vi "ASK Main.vi"() -> ()   [LabVIEW 2026]
panel:
  out "Detected Energy":dbl[](array[numeric])
  out "Recovered Binary Signal":dbl[](array[numeric])
  out "ASK Modulated Signal":dbl[](graph)
  out "Baseband Signal":dbl[](graph)
  in  "Detection Threshold":dbl
  in  "Carrier Amplitude(A)":dbl
  in  "Carrier Frequency(fc)":dbl
  in  "Bit Rate(Rb)":dbl
  in  "Sampling Frequency(Fs)":dbl
  in  "Binary Input":i32[](array[numeric])
  # ".1"
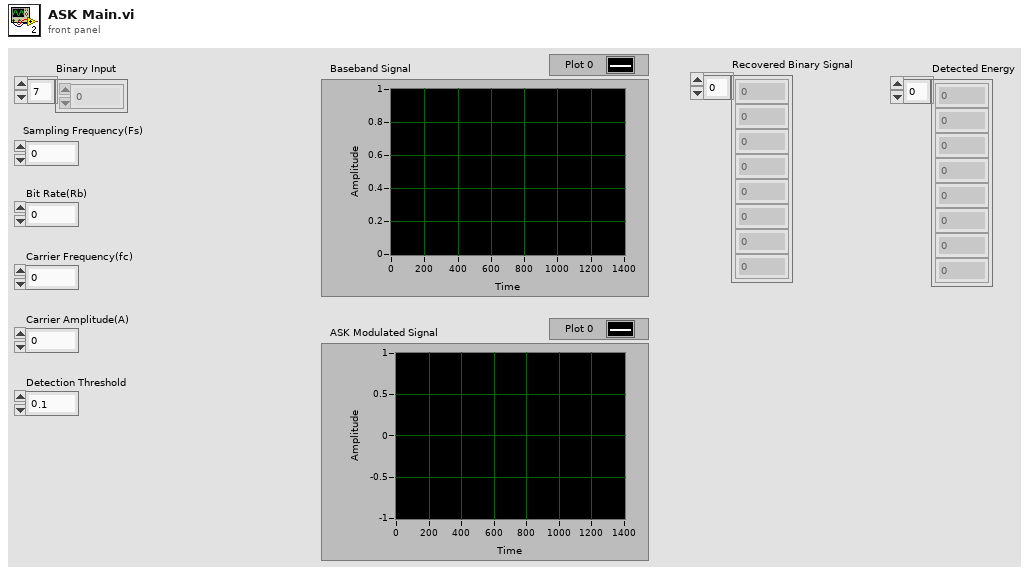
[diagram p1: front panel]
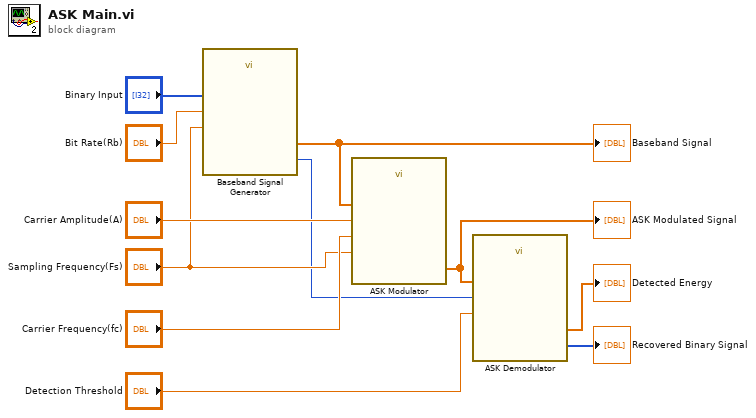
[diagram p0: block diagram]
diagram:
  n1 = call "Baseband Signal Generator.vi"("Bit Rate(Rb)"="Bit Rate(Rb)", "Sampling Frequency(Fs)"="Sampling Frequency(Fs)", "Binary Input"="Binary Input") -> ("Baseband Signal"=w9:dbl[], "Samples per bit"=w4:i32)
  "Baseband Signal" <- w9
  n2 = call "ASK Modulator.vi"("Carrier Amplitude(A)"="Carrier Amplitude(A)", "Carrier Frequency(fc)"="Carrier Frequency(fc)", "Sampling Frequency(Fs)"="Sampling Frequency(Fs)", "Baseband Signal"=w9) -> ("ASK Modulated Signal"=w5:dbl[])
  "ASK Modulated Signal" <- w5
  n3 = call "ASK Demodulator.vi"("Threshold"="Detection Threshold", "Samples per bit"=w4, "ASK Modulated Signal"=w5) -> ("Detected Energy"=→"Detected Energy":dbl[], "Recovered Binary Signal"=→"Recovered Binary Signal":i32[])
